vi "Main.vi"() -> ()   [LabVIEW 2013]
doc: "This template is for the Queued Message Handler design pattern.\n\nThe Event Handling Loop generates messages based on user interface actions.\n\nThe Message Handling Loop processes messages generated by the Event Handling Loop, or by other messages. The messages are string values, so new messages can be added easily to the Message Cases case structure in the Message Handling Loop. Each message cluster can also provide an optional value for Message Data, which is a variant that can be converted to whatever message-specific data is required."
uses:
  <vilib>/vision/Image Controls.llb/IMAQ Image.ctl
  Image Processing/Mask ROI FG Enum.ctl
  Message Passing/MsgQ Loops enum.ctl
  System Status/Status FG Enum.ctl
  Globals/Average Sector Data.vi
  controls/UI Data.ctl
  Message Queue/Message Queue.lvlib
  User Event - Stop/User Event - Stop.lvlib
  Image Processing/Image Processing.lvlib
  Common/State Machines/State Machine Lib.lvlib
  Message Passing/Main MsgQ.lvlib
  Common/GUI/GUI.lvlib
  <vilib>/rvi/interface/nirviReadWriteControl/nirviReadWriteControl.xnode
  FGs/FPGA_Reference.ctl
  FPGA Bitfiles/8-Tap8-bitCamera_FPGATarget_8-Tap8-bit_Serial_Server.lvbitx
  <vilib>/rvi/errors/niLvFpgaMergeErrorWithErrorCode.vi
  NiFpgaLv.dll
  <vilib>/rvi/errors/niLvFpgaAdjustHostInterfaceError.vi
panel:
  out "Frames Acquired":u32
  in  "Disable Background Subtraction":bool
  out "Analysis Ticks":u32
  out "Accumulate Ticks":u32
  out "FPGA Display Image":T1(plugin-control)
  out "Right Wingbeat Avg Graph":u8[](graph)
  in  "Start Serial Server":bool=TRUE
  out "Left Wingbeat Avg Graph":u8[](graph)
  in  "Stop Charts":bool
  in  "Wing ROIs":T2
  out "FPGA image info":T5={"Image Type"=0, "Unit"=enum."Undefined", "X Resolution"=2040, "Y Resolution"=1088, "X Step"=1.0, "Y Step"=1.0, "Image Name"="Image"} {"Image Type" items=["Grayscale (U8)", "Grayscale (I16)", "Grayscale (SGL)", "Complex (CSG)", "RGB (U32)", "HSL (U32)", "RGB (U64)", "Grayscale (U16)"]}
  in  "Stream?":bool
  out "FPGA Image":T1
  in  "Test Visual Response":bool
  in  "Test FPGA":bool
  out "Status Update":string="VI Stopped"
  in  "Define Mask":bool
  in  "Acquire Image":bool
  in  "Stop":bool
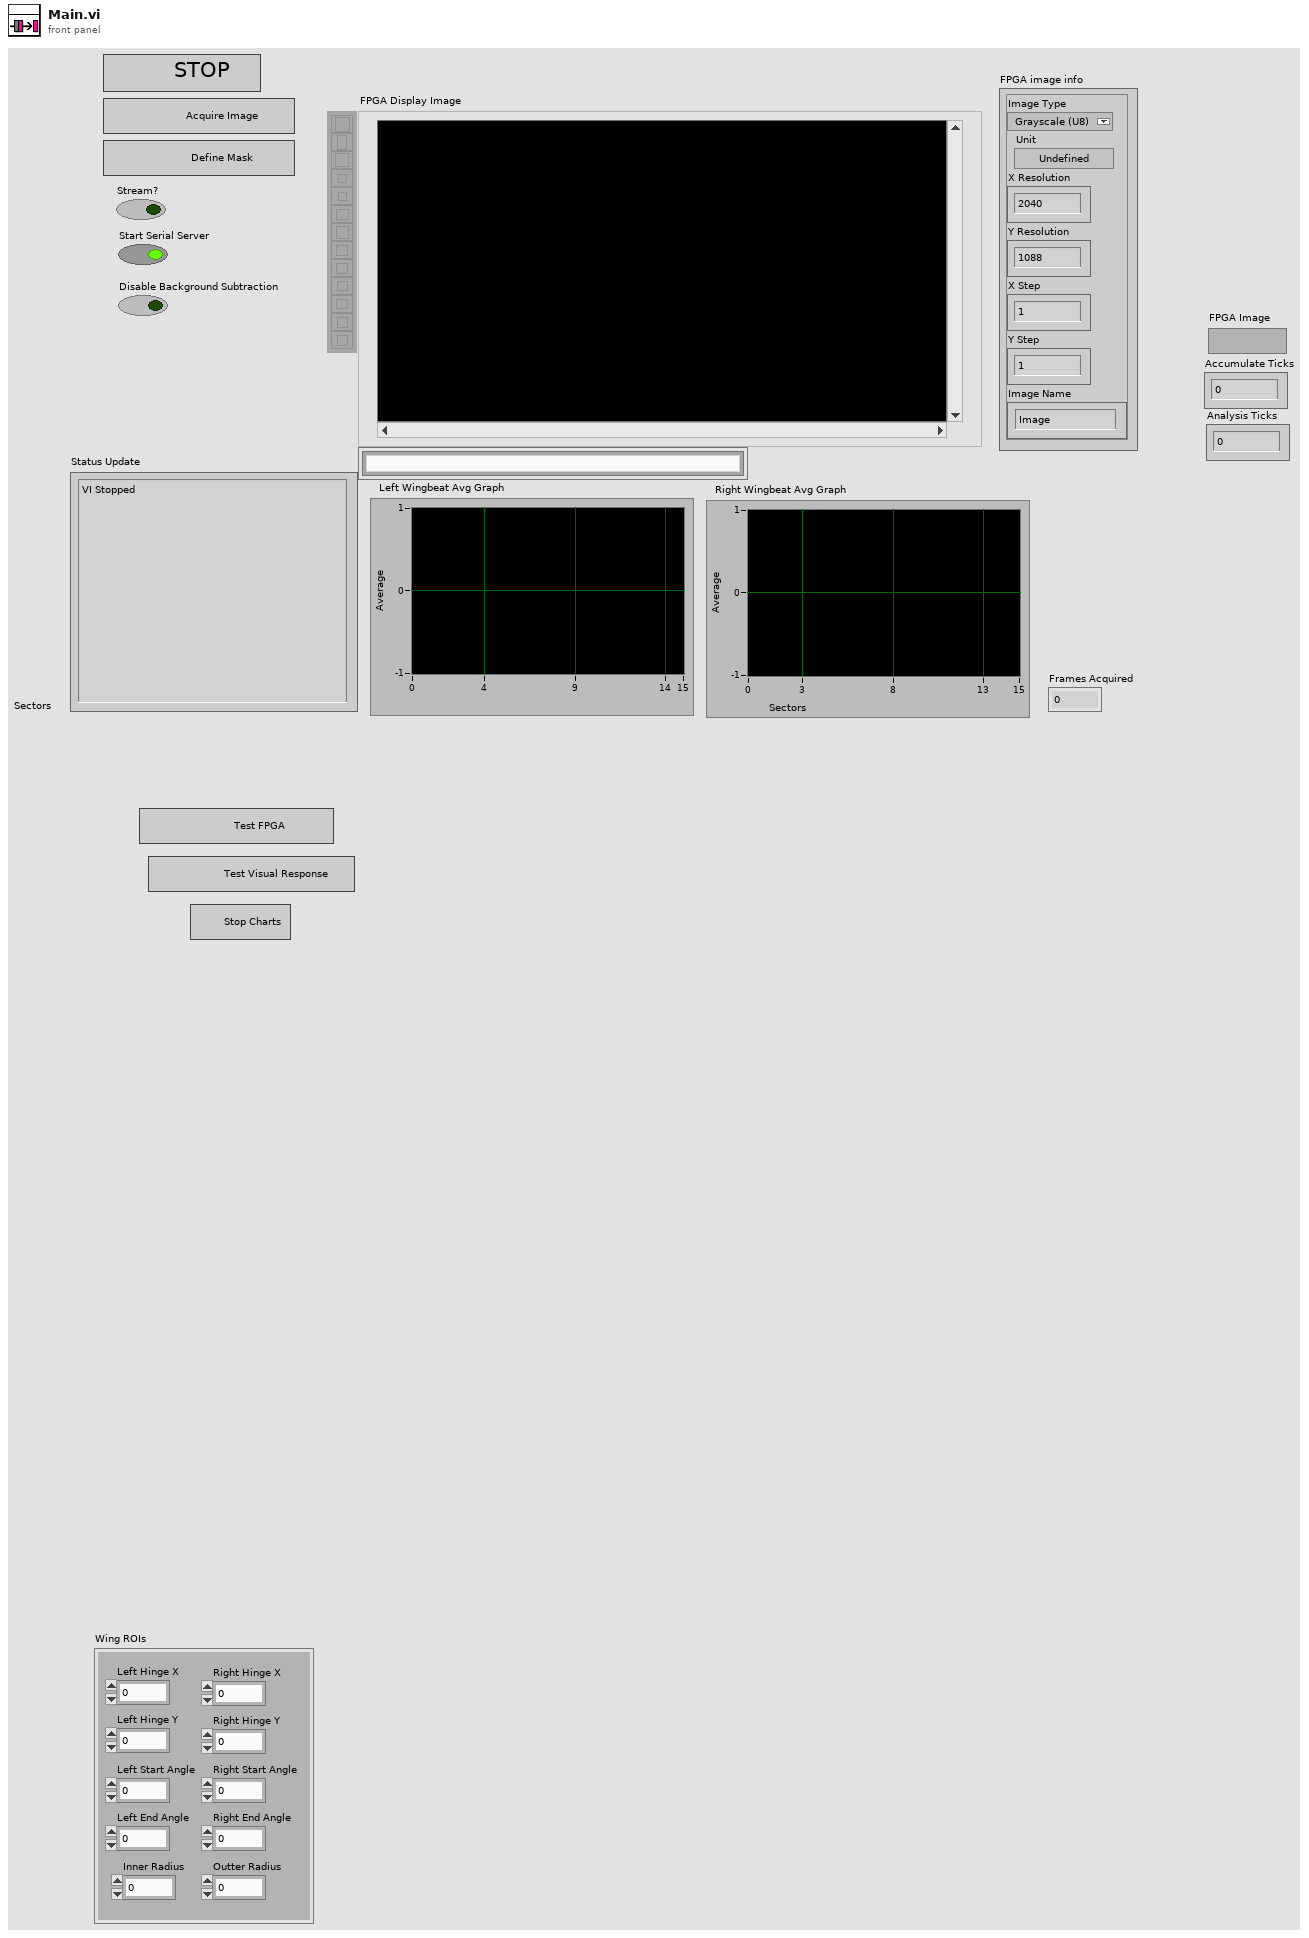
[diagram p1: front panel]
types:
  T1 = typedef "IMAQ Image.ctl" = refnum<image>
  T2 = cluster{"Left Hinge X":u16, "Left Hinge Y":u16, "Inner Radius":u16, "Outter Radius":u16, "Right Hinge X":u16, "Right Hinge Y":u16, "Right Start Angle":i16, "Right End Angle":i16, "Left Start Angle":i16, "Left End Angle":i16}
  T3 = typedef "Image Type" = u32
  T4 = typedef "Image Unit" = enum32{"Undefined", "Angström", "Micrometer", "Millimeter", "Centimeter", "Meter", "Kilometer", "Microinch", "Inch", "Feet", "Nautical miles", "Standard miles", "Steps"}
  T5 = cluster{"Image Type":T3, "Unit":T4, "X Resolution":i32, "Y Resolution":i32, "X Step":sgl, "Y Step":sgl, "Image Name":string}
  T6 = typedef "State Machine Lib.lvlib/STATE cluster.ctl" = cluster{"State":string, "Parameters":variant}
  T7 = typedef "Main MsgQ.lvlib/MsgQ Loops enum.ctl" = enum16{"User Interface", "Image Acq"}
  T8 = typedef "Mask ROI FG Enum.ctl" = enum16{"Read", "Write", "Enable Background", "Disable Background"}
  T9 = typedef "Status FG Enum.ctl" = enum16{"Reset", "Read", "Write"}
  T10 = typedef "FPGA_Reference.ctl" = refnum<k20>
  T11 = typedef "Mask ROI Cluster.ctl" = cluster{"left annulus":T12, "right annulus":T12, "Threshold Range":cluster{"Lower value":dbl, "Upper value":dbl}, "[Avg BG]":u8[], "Number of Sectors":u8, "Left ROI":T13, "Right ROI":T13, "Left Start Angle Duty Cycle":fxp<+,8,0>, "Left End Angle Duty Cycle":fxp<+,8,0>, "Right End Angle Duty Cycle":fxp<+,8,0>, "Right Start Angle Duty Cycle":fxp<+,8,0>, "[Sector ROIs]":T13[]}
  T12 = typedef "IMAQ Circle" = cluster{"Center X":i32, "Center Y":i32, "Inner Radius":i32, "Outer Radius":i32, "Start Angle":dbl, "End Angle":dbl}
  T13 = typedef "ROI Descriptor" = cluster{"Global Rectangle":i32[], "Contours":cluster{"ID":enum32{"External", "Internal"}, "Type":u32, "Coordinates":i32[]}[]}
  T14 = typedef "UI Data.ctl" = cluster{"Boolean <Replace Me>":bool, "Initial Message":string, "Numeric <Replace Me>":dbl, "Acquire Image Ref":refnum<vi>, "Define Mask Ref":refnum<vi>, "Status Update Ref":refnum<vi>, "Stop Button Ref":refnum<vi>, "FPGA Image":T1, "Processed Image":T1, "Left Annulus":cluster{"Center X":i32, "Center Y":i32, "Inner Radius":i32, "Outer Radius":i32, "Start Angle":dbl, "End Angle":dbl}, "Right Annulus":cluster{"Center X":i32, "Center Y":i32, "Inner Radius":i32, "Outer Radius":i32, "Start Angle":dbl, "End Angle":dbl}}
  T15 = typedef "Message Queue.lvlib/All Message Queues.ctl" = cluster{"UI":refnum<queue>}
  T16 = cluster{"Center X":i32, "Center Y":i32, "Inner Radius":i32, "Outer Radius":i32, "Start Angle":dbl, "End Angle":dbl}
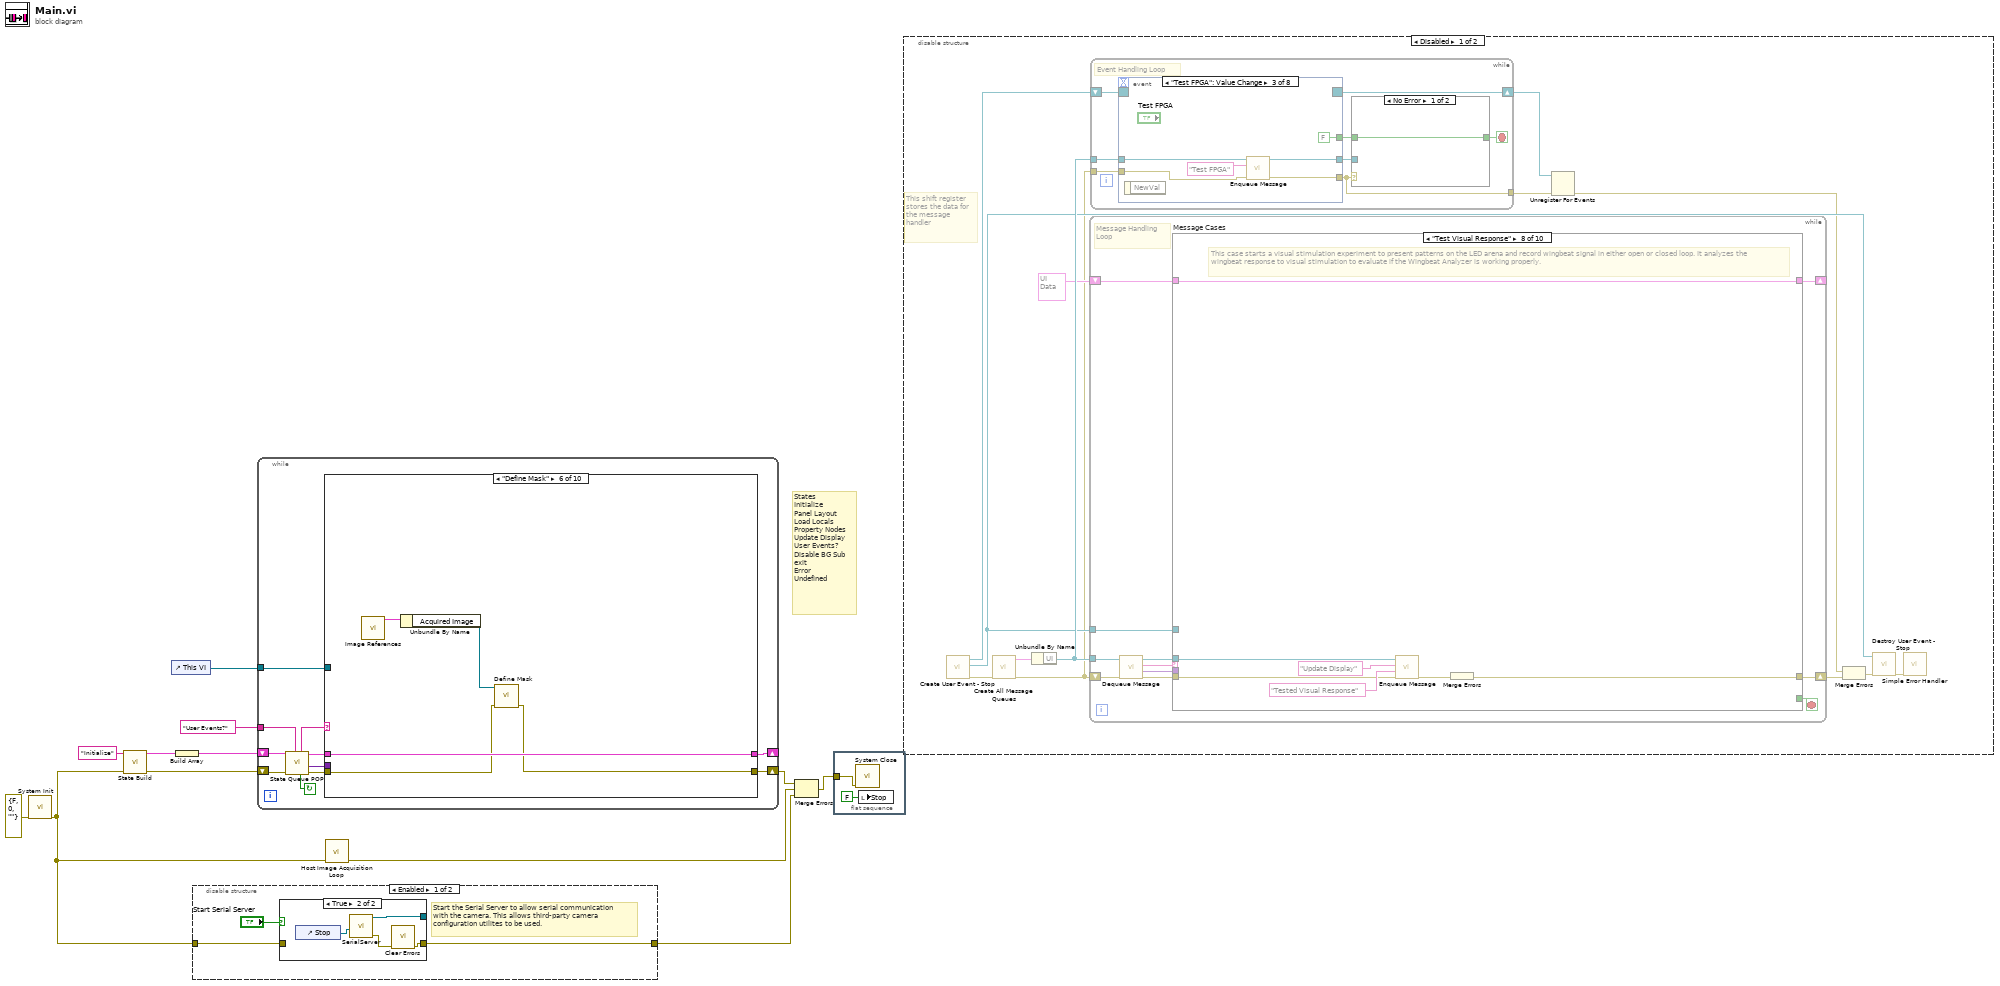
[diagram p0: block diagram]
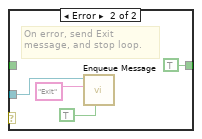
[diagram p4: hidden frame]
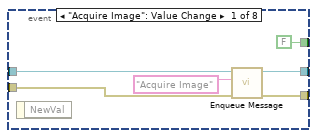
[diagram p5: hidden frame]
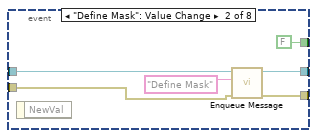
[diagram p6: hidden frame]
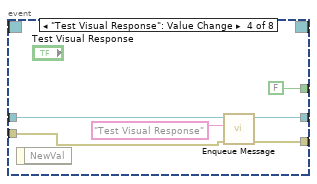
[diagram p7: hidden frame]
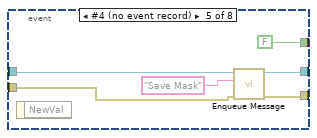
[diagram p8: hidden frame]
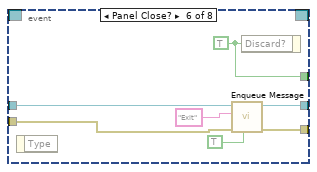
[diagram p9: hidden frame]
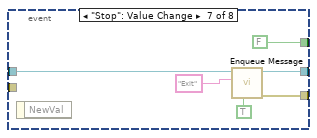
[diagram p10: hidden frame]
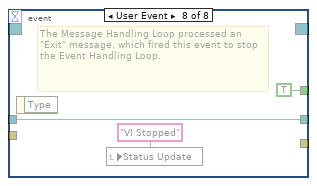
[diagram p11: hidden frame]
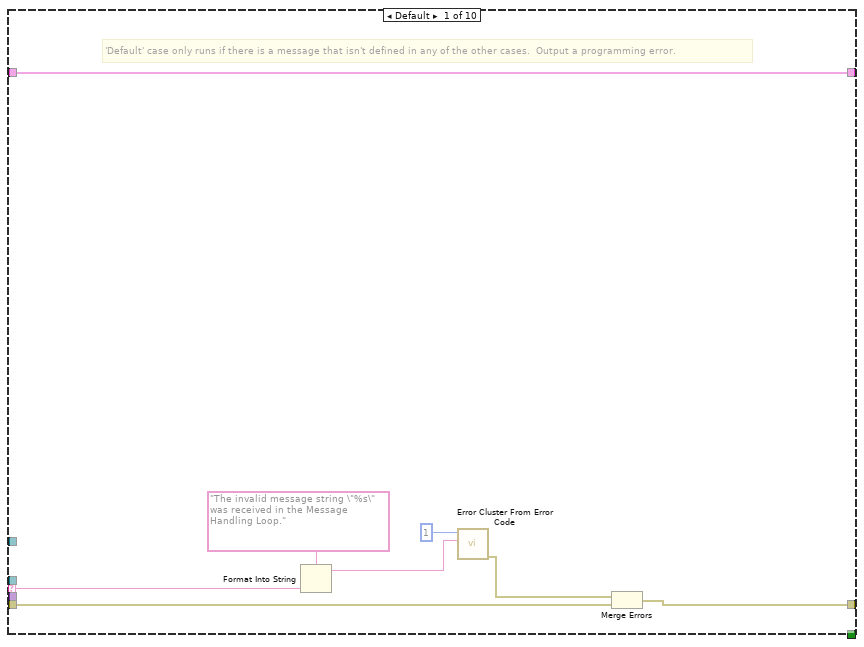
[diagram p12: hidden frame]
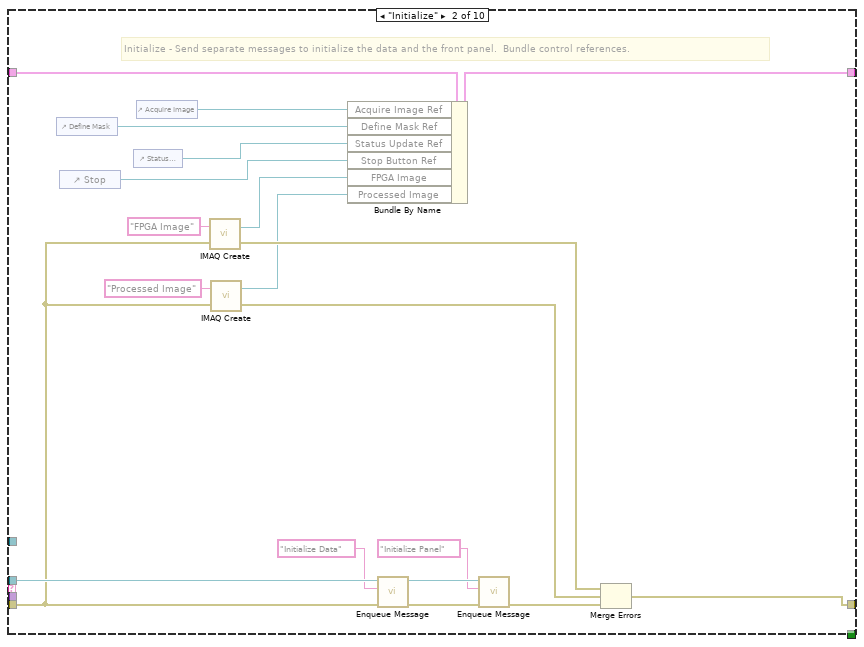
[diagram p13: hidden frame]
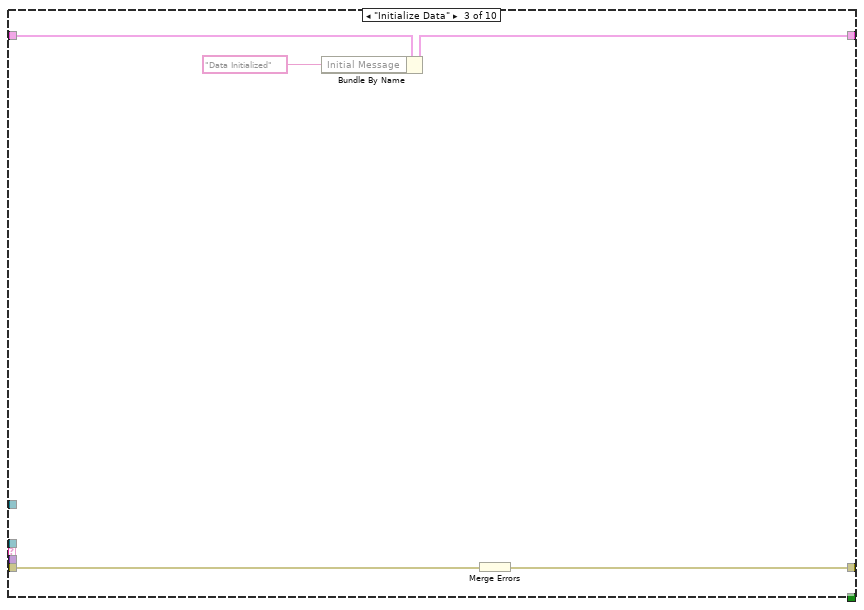
[diagram p14: hidden frame]
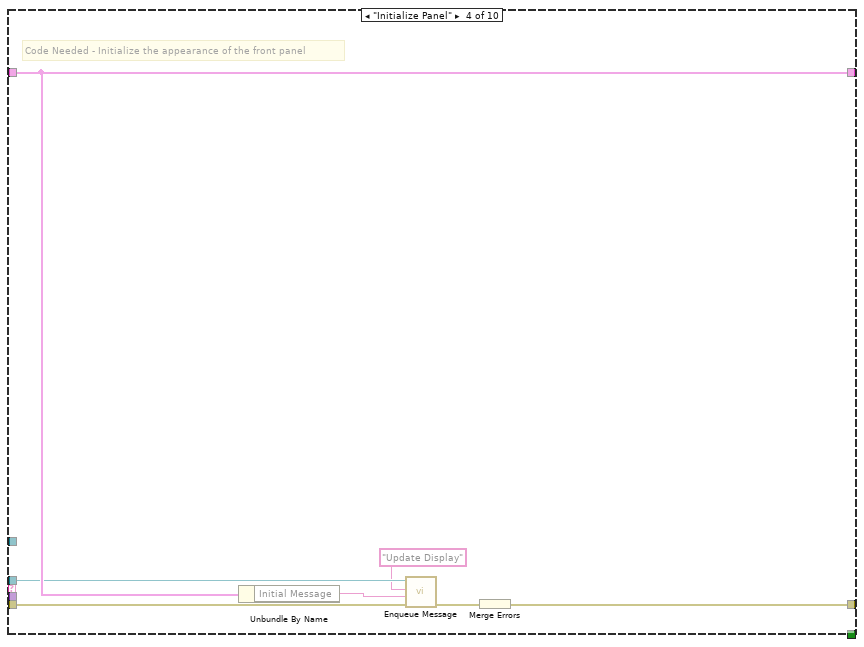
[diagram p15: hidden frame]
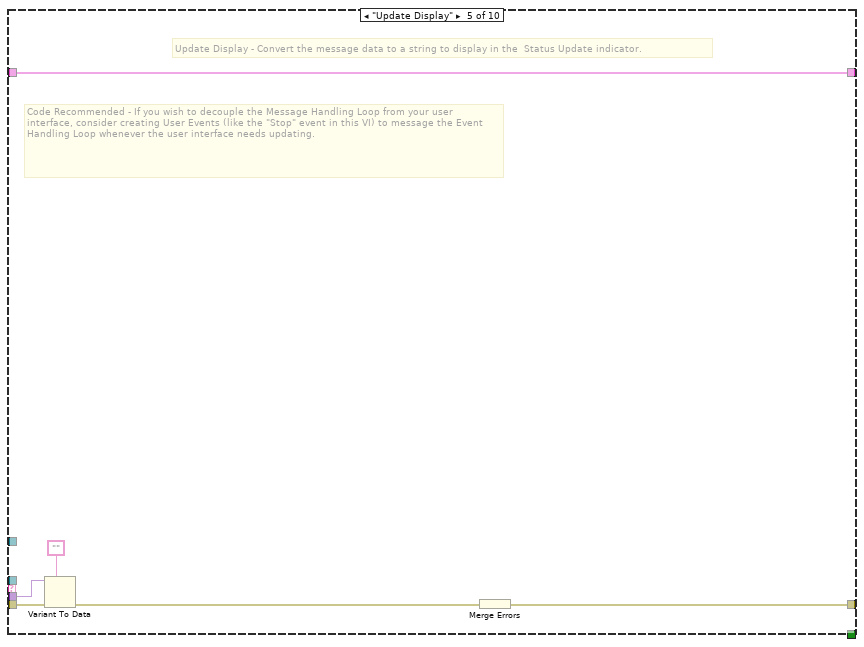
[diagram p16: hidden frame]
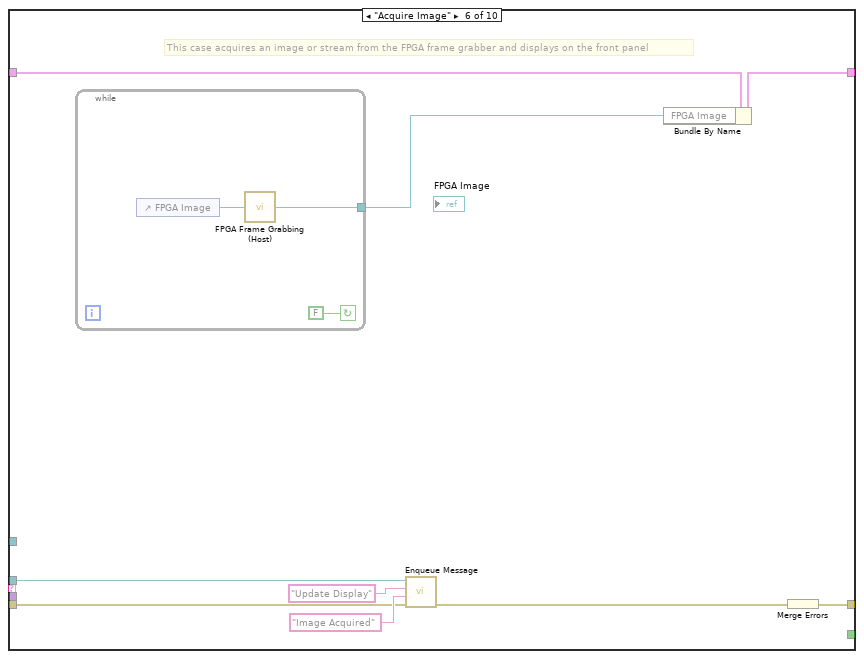
[diagram p17: hidden frame]
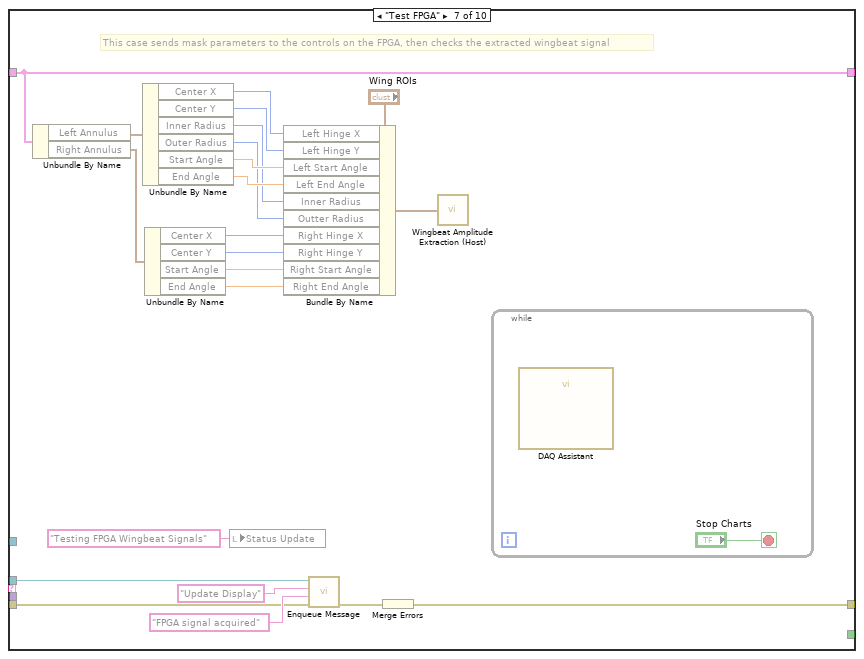
[diagram p18: hidden frame]
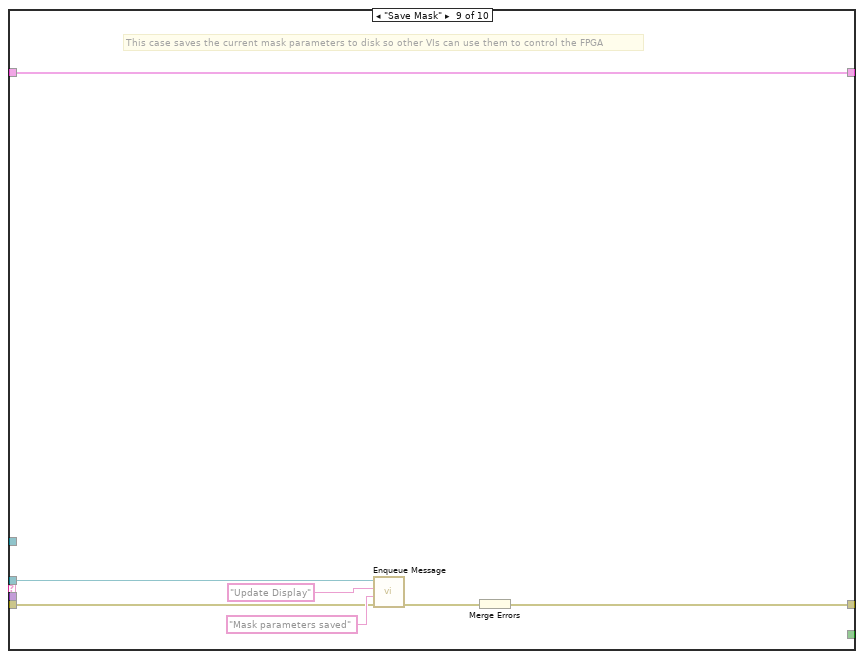
[diagram p19: hidden frame]
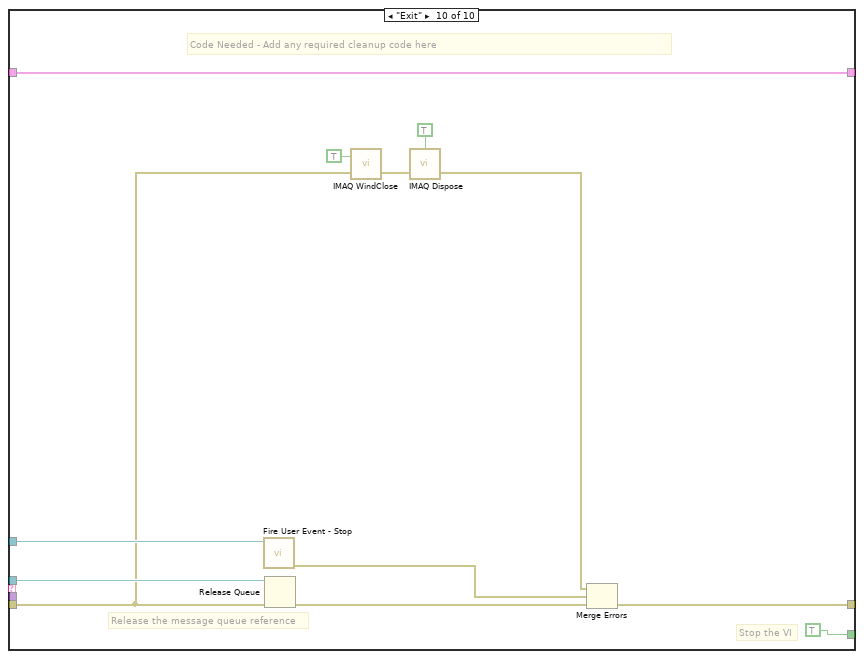
[diagram p20: hidden frame]
diagram:
  # "States\nInitialize\nPanel Layout\nLoad Locals\nProperty Nodes\nUpdate Display\nUser Events?\nDisable BG Sub\nexit\nError\nUndefined"
  n1 = call "System Init.vi"("error in (no error)"=errorcluster {"status"=FALSE, "code"=0, "source"=""}) -> ("error out"=w11:errorcluster)  [unwired: 10 in]
  n2 = call "State Build.vi"("error in (no error)"=w11, "State"="Initialize") -> ("error out"=w7:errorcluster, "State Out"=w9:T6)  [unwired: 8 in]
  n3 = control-ref of="This VI"() -> (w5:refnum<vi>)
  n4 = Build Array(w9) -> (w8:T6[])
  n5 = disable-structure shown="Enabled" {
    disable-tunnel: w11 -> [w14 _]
    disable-tunnel: [w13 _] -> w1
    frame Enabled {
      # "Start the Serial Server to allow serial communication\nwith the camera. This allows third-party camera\nconfiguration utilites to be used."
      n6 = case shown="True" "Start Serial Server" {
        tunnel: [_ w20] -> _
        tunnel: w14 -> [w16 _]
        tunnel: [w16 w18] -> w13
        frame False {
        }
        frame True {
          n7 = control-ref of="Stop"() -> (w19:refnum<vi>)
          n8 = call "SerialServer.vi"("Stop Refnum"=w19) -> ("error out"=w17:errorcluster, "FPGA VI Reference Out"=w20:refnum<k20>)  [unwired: 5 in]
          n9 = call <vilib>:"Clear Errors.vi"("error in (no error)"=w17) -> ("error out"=w18:errorcluster)  [unwired: 6 in]
        }
      }
    }
    frame Disabled {
    }
  }
  n10 = while {
    shift-right: [w25] -> _
    shift-left: w8 -> [w31]
    shift-right: [w23] -> w4
    shift-left: w7 -> [w30]
    tunnel: "User Events?" ("State") -> [w28]
    tunnel: w5 -> [w26]
    stop <- w29 continue-if-true
    n11 = call "State Queue POP.vi"("Default state"=w28, "error in (no error)"=w30, "State que in"=w31) -> ("error out"=w22:errorcluster, "Parameters"=w21:variant, "State que out"=w24:T6[], "Not Exit?"=w29:bool, "State case out"=w27:string)  [unwired: 4 in]
    n12 = case shown="\"Define Mask\"" w27 {
      tunnel: w26 -> [_ _ w42 _ _ _ _ _ _ _]
      tunnel: [w33 w34 w39 w45 w47 w52 w53 w70 w108 w136] -> w25
      tunnel: w24 -> [w33 w37 w39 w45 w47 w52 w53 w69 _ w136]
      tunnel: [w32 w35 w40 w44 w46 w50 w54 w68 w107 w134] -> w23
      tunnel: w22 -> [w32 w36 w41 w44 w46 w51 w65 w67 w109 w118]
      tunnel: w21 -> [_ _ _ _ _ _ w64 w66 _ _]
      frame Default {
      }
      frame "Initialize" {
        n13 = call "State Queue PUSH multiple states no parameters.vi"("States to queue"=string[] ["Panel Layout", "Load Locals", "Property Nodes", "Update Display"], "error in (no error)"=w36, "State que in"=w37) -> ("error out"=w35:errorcluster, "State que out"=w34:T6[])  [unwired: 7 in]
      }
      frame "Panel Layout" {
        # "Reset origin to 0,0"
        n14 = call "Reset all pane origins.vi"("error in (no error"=w41, "Vi Ref In"=w42) -> ("error out"=w40:errorcluster)  [unwired: 8 in, 1 out]
      }
      frame "Load Locals" {
        w43 = FALSE ("Stream?")
        n15 = local write "Stream?"(w43) -> ()
        n16 = local write "Disable Background Subtraction"(w43) -> ()
      }
      frame "Property Nodes" {
      }
      frame "Define Mask" {
        n17 = call "Image References.vi"() -> ("Images"=w49:cluster{"Acquired Image":T1, "Display Image":T1})  [unwired: 10 in, 1 out]
        n18 = Unbundle By Name(w49) -> ("Acquired Image"=w48:T1)
        n19 = call "Define Mask.vi"("error in (no error)"=w51, "FPGA Image"=w48) -> ("error out"=w50:errorcluster)  [unwired: 9 in]
      }
      frame "Disable BG Sub" {
        n20 = Variant To Data(error in=w65, type=FALSE, Variant=w64) -> (data=w62:bool, error out=w59:errorcluster)
        n21 = Select(t=Mask_ROI_FG_Enum."Disable Background" ("Operation"), s=w62, f=Mask_ROI_FG_Enum."Enable Background" ("Operation")) -> (s? t:f=w58:T8)
        n22 = call "Mask ROI FG.vi"("error in (no error)"=w59, "Operation"=w58) -> ("error out"=w55:errorcluster)  [unwired: 8 in, 1 out]
        n23 = call "Send MsgQ.vi"("error in (no error)"=w55, "Message String"="Update Sector Parameters", "Send to MsgQ"=MsgQ_Loops_enum."Image Acq") -> ("error out"=w54:errorcluster)  [unwired: 8 in]
      }
      frame "User Events?" {
        n24 = event shown="[0] Timeout" {
          selector: _ -> [_ _ _ _ _ _]
          dyn-events: _ -> [_ _ _ _ _ _]
          timeout: 200 -> [_ _ _ _ _ _]
          tunnel: [w73 w83 w86 w93 w99 w102] -> w70
          tunnel: w69 -> [w74 w83 w86 w95 w101 w105]
          tunnel: [w75 w80 w87 w92 w98 w103] -> w68
          tunnel: w67 -> [w76 w81 w88 w94 w100 w104]
          tunnel: w66 -> [_ _ _ _ _ _]
          event Timeout {
            n25 = event-data() -> ()  [unwired: 1 in, 3 out]
            n26 = disable-structure shown="Disabled" {
              frame Disabled {
                n27 = call "FPGA Reference FG.vi"() -> ("FPGA VI Reference Out"=w79:T10)  [unwired: 11 in]
                n28 = xnode "Read/Write Control"("FPGA VI Reference In"=w79) -> ("Accumulate Ticks"=→"Accumulate Ticks", "Analysis Ticks"=→"Analysis Ticks":u32)  [unwired: 1 in, 2 out]
              }
              frame Enabled {
              }
            }
            n29 = call "State Queue PUSH.vi"("State case"="Update Display", "error in (no error)"=w76, "State que in"=w74) -> ("error out"=w75:errorcluster, "State que out"=w73:T6[])  [unwired: 7 in]
          }
          event "Acquire Image": Value Change {
            n30 = event-data() -> ()  [unwired: 1 in, 6 out]
            n31 = call "Send MsgQ.vi"("error in (no error)"=w81, "Message String"="Acquire Single Image", "Send to MsgQ"=MsgQ_Loops_enum."Image Acq") -> ("error out"=w80:errorcluster)  [unwired: 8 in]
          }
          event "Stream?": Value Change {
            n32 = event-data() -> ("NewVal"=w85:bool)  [unwired: 1 in, 5 out]
            n33 = call "Send MsgQ.vi"("error in (no error)"=w88, "Data In"=w85, "Message String"="Stream Image", "Send to MsgQ"=MsgQ_Loops_enum."Image Acq") -> ("error out"=w87:errorcluster)  [unwired: 7 in]
          }
          event "Define Mask": Value Change {
            n34 = event-data() -> ()  [unwired: 1 in, 6 out]
            n35 = call "State Queue PUSH.vi"("State case"="Define Mask", "error in (no error)"=w94, "State que in"=w95) -> ("error out"=w92:errorcluster, "State que out"=w93:T6[])  [unwired: 7 in]
          }
          event "Disable Background Subtraction": Value Change {
            n36 = event-data() -> ("NewVal"=w96:bool)  [unwired: 1 in, 5 out]
            n37 = call "State Queue PUSH.vi"("State case"="Disable BG Sub", "error in (no error)"=w100, "Parameters"=w96, "State que in"=w101) -> ("error out"=w98:errorcluster, "State que out"=w99:T6[])  [unwired: 6 in]
          }
          event "Stop": Value Change {
            n38 = event-data() -> ()  [unwired: 1 in, 6 out]
            n39 = call "State Queue PUSH.vi"("State case"="exit", "error in (no error)"=w104, "State que in"=w105) -> ("error out"=w103:errorcluster, "State que out"=w102:T6[])  [unwired: 7 in]
          }
        }
      }
      frame "exit" {
        n40 = call "Broadcast Exit.vi"("error in"=w109) -> ("error out"=w107:errorcluster)  [unwired: 10 in]
        n41 = call "Queue EXIT state.vi"() -> ("Exit State Q"=w108:T6[])  [unwired: 1 in]
      }
      frame "Update Display" {
        n42 = call "Image References.vi"() -> ("Images"=w114:cluster{"Acquired Image":T1, "Display Image":T1})  [unwired: 10 in, 1 out]
        n43 = call "Status FG.vi"("Operation"=Status_FG_Enum."Read") -> ("Status Out"=→"Status Update":string)  [unwired: 9 in, 1 out]
        n44 = call "Mask ROI FG.vi"("Operation"=Mask_ROI_FG_Enum."Read") -> ("Mask ROI Out"=w131:T11)  [unwired: 9 in, 1 out]
        n45 = Unbundle By Name(w114) -> ("Acquired Image"=w113:T1, "Display Image"=w112:T1)
        n46 = Unbundle By Name(w131) -> ("Number of Sectors"=w128:u8)
        n47 = global read "Average Sector Data.vi" "# of Frames Acquired"() -> (→"Frames Acquired":u32)
        n48 = global read "Average Sector Data.vi" "[Average Sector Data]"() -> (w133:u8[])
        n49 = call "Overlay Image with Sector ROI.vi"("FPGA Display Image In"=w112, "error in"=w118, "FPGA Image"=w113) -> ("error out"=w117:errorcluster, "FPGA Display Image Out"=→"FPGA Display Image":T1)  [unwired: 7 in]
        n50 = call "IMAQ GetImageInfo"("error in (no error)"=w117, "Image"=w113) -> ("error out"=w135:errorcluster, "X Step"=w123:sgl, "Y Resolution"=w122:i32, "X Resolution"=w121:i32, "Y Step"=w124:sgl, "Unit"=w120:T4, "Image Name"=w125:string, "Image Type"=w119:T3)  [unwired: 2 in]
        n51 = Split 1D Array(array=w133, index=w128) -> (first subarray=→"Left Wingbeat Avg Graph":u8[], second subarray=→"Right Wingbeat Avg Graph":u8[])
        n52 = local read "FPGA image info"() -> (w127:T5)
        n53 = Bundle By Name(cluster=w127, "Image Type"=w119, "Unit"=w120, "X Resolution"=w121, "Y Resolution"=w122, "X Step"=w123, "Y Step"=w124, "Image Name"=w125) -> (→"FPGA image info":T5)
        n54 = call <vilib>:"Clear Errors.vi"("error in (no error)"=w135) -> ("error out"=w134:errorcluster)  [unwired: 6 in]
      }
    }
  }
  n55 = call "Host Image Acquisition Loop.vi"("error in"=w11) -> ("error out"=w3:errorcluster)  [unwired: 10 in]
  n56 = Merge Errors(w4, w3, w1) -> (w2:errorcluster)
  n57 = flat-sequence {
    tunnel: w2 -> [w138]
    frame #0 {
      n58 = call "System Close.vi"("error in (no error)"=w138) -> ()  [unwired: 10 in, 1 out]
      n59 = local write "Stop"(FALSE ("Stop")) -> ()
    }
  }
  n60 = disable-structure shown="Disabled" {
    frame Disabled {
      # "This shift register\nstores the data for the message handler"
      n61 = call "Create User Event - Stop.vi"() -> ("error out"=w147:errorcluster, "User Event - Stop"=w144:refnum<user-event>, "Stop Event Registration Refnum"=w148:refnum<event-registration>)  [unwired: 9 in]
      n62 = call "Create All Message Queues.vi"("error in (no error)"=w147) -> ("error out"=w139:errorcluster, "Message Queues out"=w151:T15)  [unwired: 9 in]
      n63 = Unbundle By Name(w151) -> ("UI"=w149:refnum<queue>)
      n64 = while {
        tunnel: w149 -> [w211]
        shift-right: [w220] -> _
        shift-left: T14 {"Boolean <Replace Me>"=TRUE, "Initial Message"="", "Numeric <Replace Me>"=0.0, "Acquire Image Ref"=refnum, "Define Mask Ref"=refnum, "Status Update Ref"=refnum, "Stop Button Ref"=refnum, "FPGA Image"=refnum, "Processed Image"=refnum, "Left Annulus"={"Center X"=0, "Center Y"=0, "Inner Radius"=0, "Outer Radius"=0, "Start Angle"=0.0, "End Angle"=0.0}, "Right Annulus"={"Center X"=0, "Center Y"=0, "Inner Radius"=0, "Outer Radius"=0, "Start Angle"=0.0, "End Angle"=0.0}} ("Data Cluster") -> [w221]
        tunnel: w144 -> [w217]
        shift-right: [w218] -> w150
        shift-left: w139 -> [w216]
        stop <- w219 stop-if-true
        # "Message Handling Loop"
        n65 = call "Dequeue Message.vi"("error in (no error)"=w216, "Message Queue"=w211) -> ("error out"=w215:errorcluster, "Message Data"=w213:variant, "Message"=w214:string, "dup Message Queue"=w212:refnum<queue>)  [unwired: 6 in]
        n66 = case "Message Cases" shown="\"Test Visual Response\"" w214 {
          selector: w214 -> [w227 _ _ _ _ _ _ _ _ _]
          tunnel: w212 -> [_ w247 _ w258 _ w275 w298 w306 w314 w330]
          tunnel: w215 -> [w224 w232 w254 w259 w266 w270 w299 w307 w312 w319]
          tunnel: [w222 w234 w250 w260 w267 w277 w297 w305 w317 w326] -> w218
          tunnel: w221 -> [w229 w244 w253 w261 w268 w272 w296 w311 w318 w329]
          tunnel: [w229 w243 w252 w261 w268 w271 w296 w311 w318 w329] -> w220
          tunnel: [_ _ _ _ _ _ _ _ _ TRUE] -> w219
          tunnel: w213 -> [_ _ _ _ w265 _ _ _ _ _]
          tunnel: w217 -> [_ _ _ _ _ _ _ _ _ w325]
          frame Default {
            # "'Default' case only runs if there is a message that isn't defined in any of the other cases.  Output a programming error."
            n67 = Format Into String(format string="The invalid message string \"%s\" was received in the Message Handling Loop." ("Unknown Message Error Text"), w227) -> (resulting string=w225:string)  [unwired: 2 in, 1 out]
            n68 = call <vilib>:"Error Cluster From Error Code.vi"("error message (\"\")"=w225, "error code (0)"=1) -> ("error out"=w223:errorcluster)  [unwired: 7 in]
            n69 = Merge Errors(w223, w224) -> (w222:errorcluster)
          }
          frame "Initialize" {
            # "Initialize - Send separate messages to initialize the data and the front panel.  Bundle control references."
            n70 = control-ref of="Define Mask"() -> (w241:refnum<vi>)
            n71 = control-ref of="Stop"() -> (w239:refnum<vi>)
            n72 = control-ref of="Status Update"() -> (w240:refnum<vi>)
            n73 = control-ref of="Acquire Image"() -> (w242:refnum<vi>)
            n74 = call "IMAQ Create"("Image Name"="FPGA Image", "error in (no error)"=w232) -> ("New Image"=w237:T1, "error out"=w233:errorcluster)  [unwired: 3 in]
            n75 = call "IMAQ Create"("Image Name"="Processed Image", "error in (no error)"=w232) -> ("New Image"=w230:T1, "error out"=w231:errorcluster)  [unwired: 3 in]
            n76 = Bundle By Name(cluster=w244, "Acquire Image Ref"=w242, "Define Mask Ref"=w241, "Status Update Ref"=w240, "Stop Button Ref"=w239, "FPGA Image"=w237, "Processed Image"=w230) -> (w243:T14)
            n77 = call "Enqueue Message.vi"("error in (no error)"=w232, "Message"="Initialize Data", "Message Queue"=w247) -> ("error out"=w249:errorcluster, "dup Message Queue"=w248:refnum<queue>)  [unwired: 7 in]
            n78 = call "Enqueue Message.vi"("error in (no error)"=w249, "Message"="Initialize Panel", "Message Queue"=w248) -> ("error out"=w235:errorcluster)  [unwired: 7 in, 1 out]
            n79 = Merge Errors(w233, w231, w235) -> (w234:errorcluster)
          }
          frame "Initialize Data" {
            n80 = Bundle By Name(cluster=w253, "Initial Message"="Data Initialized") -> (w252:T14)
            n81 = Merge Errors(w254) -> (w250:errorcluster)
          }
          frame "Initialize Panel" {
            # "Code Needed - Initialize the appearance of the front panel"
            n82 = Unbundle By Name(w261) -> ("Initial Message"=w255:string)
            n83 = call "Enqueue Message.vi"("error in (no error)"=w259, "Message Data"=w255, "Message"="Update Display", "Message Queue"=w258) -> ("error out"=w257:errorcluster)  [unwired: 6 in, 1 out]
            n84 = Merge Errors(w257) -> (w260:errorcluster)
          }
          frame "Update Display" {
            # "Code Recommended - If you wish to decouple the Message Handling Loop from your user interface, consider creating User Events (like the \"Stop\" event in this VI) to message the Event Handling Loop whenever the user interface needs updating."
            # "Update Display - Convert the message data to a string to display in the  Status Update indicator."
            n85 = Variant To Data(error in=w266, type="", Variant=w265) -> (data=w262:string, error out=w263:errorcluster)
            n86 = Merge Errors(w263) -> (w267:errorcluster)
          }
          frame "Acquire Image" {
            # "This case acquires an image or stream from the FPGA frame grabber and displays on the front panel"
            n87 = while {
              tunnel: [w280] -> w269
              stop <- FALSE continue-if-true
              n88 = control-ref of="FPGA Image"() -> (w279:refnum<vi>)
              n89 = call "FPGA Frame Grabbing (Host).vi"("Ctl Refnum"=w279) -> ("Image"=w280:T1)
            }
            n90 = call "Enqueue Message.vi"("error in (no error)"=w270, "Message Data"="Image Acquired" ("\"Do Something\" button pressed"), "Message"="Update Display", "Message Queue"=w275) -> ("error out"=w276:errorcluster)  [unwired: 6 in, 1 out]
            n91 = Bundle By Name(cluster=w272, "FPGA Image"=w269) -> (w271:T14)
            n92 = Merge Errors(w276) -> (w277:errorcluster)
          }
          frame "Test FPGA" {
            # "This case sends mask parameters to the controls on the FPGA, then checks the extracted wingbeat signal"
            n93 = Unbundle By Name(w296) -> ("Left Annulus"=w295:T16, "Right Annulus"=w294:T16)
            n94 = Unbundle By Name(w295) -> ("Center X"=w292:i32, "Center Y"=w291:i32, "Inner Radius"=w288:i32, "Outer Radius"=w287:i32, "Start Angle"=w290:dbl, "End Angle"=w289:dbl)
            n95 = Unbundle By Name(w294) -> ("Center X"=w286:i32, "Center Y"=w285:i32, "Start Angle"=w284:dbl, "End Angle"=w283:dbl)
            n96 = local write "Status Update"("Testing FPGA Wingbeat Signals" ("Status Update")) -> ()
            n97 = Bundle By Name(cluster="Wing ROIs", "Left Hinge X"=w292, "Left Hinge Y"=w291, "Left Start Angle"=w290, "Left End Angle"=w289, "Inner Radius"=w288, "Outter Radius"=w287, "Right Hinge X"=w286, "Right Hinge Y"=w285, "Right Start Angle"=w284, "Right End Angle"=w283) -> (w282:T2)
            n98 = call "Enqueue Message.vi"("error in (no error)"=w299, "Message Data"="FPGA signal acquired" ("\"Do Something\" button pressed"), "Message"="Update Display", "Message Queue"=w298) -> ("error out"=w302:errorcluster)  [unwired: 6 in, 1 out]
            n99 = Merge Errors(w302) -> (w297:errorcluster)
            n100 = call "Wingbeat Amplitude Extraction (Host).vi"("Wing ROIs"=w282) -> ()  [unwired: 1 in]
            n101 = while {
              stop <- "Stop Charts" stop-if-true
              n102 = call "DAQ Assistant"() -> ("data"=w303:dynamicdata)  [unwired: 17 in, 2 out]
            }
          }
          frame "Test Visual Response" {
            # "This case starts a visual stimulation experiment to present patterns on the LED arena and record wingbeat signal in either open or closed loop. It analyzes the wingbeat response to visual stimulation to evaluate if the Wingbeat Analyzer is working properly."
            n103 = call "Enqueue Message.vi"("error in (no error)"=w307, "Message Data"="Tested Visual Response" ("\"Do Something\" button pressed"), "Message"="Update Display", "Message Queue"=w306) -> ("error out"=w310:errorcluster)  [unwired: 6 in, 1 out]
            n104 = Merge Errors(w310) -> (w305:errorcluster)
          }
          frame "Save Mask" {
            # "This case saves the current mask parameters to disk so other VIs can use them to control the FPGA"
            n105 = call "Enqueue Message.vi"("error in (no error)"=w312, "Message Data"="Mask parameters saved" ("\"Do Something Else\" button pressed"), "Message"="Update Display", "Message Queue"=w314) -> ("error out"=w313:errorcluster)  [unwired: 6 in, 1 out]
            n106 = Merge Errors(w313) -> (w317:errorcluster)
          }
          frame "Exit" {
            # "Stop the VI"
            # "Release the message queue reference"
            # "Code Needed - Add any required cleanup code here"
            n107 = call "Fire User Event - Stop.vi"("User Event - Stop"=w325) -> ("error out"=w324:errorcluster)  [unwired: 10 in]
            n108 = Release Queue(queue=w330, error in (no error)=w319) -> (error out=w327:errorcluster)  [unwired: 1 in, 2 out]
            n109 = call "IMAQ WindClose"("Close All Windows (False)"=TRUE, "error in (no error)"=w319) -> ("error out"=w321:errorcluster)  [unwired: 4 in]
            n110 = call "IMAQ Dispose"("All Images? (No)"=TRUE, "error in (no error)"=w321) -> ("error out"=w320:errorcluster)  [unwired: 4 in]
            n111 = Merge Errors(w320, w324, w327) -> (w326:errorcluster)
          }
        }
      }
      n112 = while {
        tunnel: w149 -> [w159]
        tunnel: [w155] -> w142
        shift-right: [w153] -> w141
        shift-left: w148 -> [w154]
        tunnel: w139 -> [w152]
        stop <- w157 stop-if-true
        # "Event Handling Loop"
        n113 = event shown="[2] \"Test FPGA\": Value Change" {
          selector: w154 -> [_ _ _ _ _ _ _ _]
          dyn-events: [_ _ _ _ _ _ _ _] -> w153
          timeout: _ -> [_ _ _ _ _ _ _ _]
          tunnel: [FALSE ("Discard?") FALSE ("Discard?") FALSE ("Discard?") FALSE ("Discard?") FALSE ("Discard?") w201 FALSE ("Discard?") TRUE ("Discard?")] -> w158
          tunnel: w159 -> [w170 w176 w182 w187 w192 w200 w207 w210]
          tunnel: [w169 w174 w179 w184 w189 w199 w206 _] -> w155
          tunnel: [w168 w175 w178 w186 w191 w198 w204 w210] -> w156
          tunnel: w152 -> [w166 w172 w180 w183 w190 w195 _ _]
          event "Acquire Image": Value Change {
            n114 = event-data() -> ()  [unwired: 1 in, 1 out]
            n115 = call "Enqueue Message.vi"("error in (no error)"=w166, "Message"="Acquire Image", "Message Queue"=w170) -> ("error out"=w169:errorcluster, "dup Message Queue"=w168:refnum<queue>)  [unwired: 7 in]
          }
          event "Define Mask": Value Change {
            n116 = event-data() -> ()  [unwired: 1 in, 1 out]
            n117 = call "Enqueue Message.vi"("error in (no error)"=w172, "Message"="Define Mask", "Message Queue"=w176) -> ("error out"=w174:errorcluster, "dup Message Queue"=w175:refnum<queue>)  [unwired: 7 in]
          }
          event "Test FPGA": Value Change {
            n118 = event-data() -> ()  [unwired: 1 in, 1 out]
            n119 = call "Enqueue Message.vi"("error in (no error)"=w180, "Message"="Test FPGA", "Message Queue"=w182) -> ("error out"=w179:errorcluster, "dup Message Queue"=w178:refnum<queue>)  [unwired: 7 in]
          }
          event "Test Visual Response": Value Change {
            n120 = event-data() -> ()  [unwired: 1 in, 1 out]
            n121 = call "Enqueue Message.vi"("error in (no error)"=w183, "Message"="Test Visual Response", "Message Queue"=w187) -> ("error out"=w184:errorcluster, "dup Message Queue"=w186:refnum<queue>)  [unwired: 7 in]
          }
          event #4 (no event record) {
            n122 = event-data() -> ()  [unwired: 1 in, 1 out]
            n123 = call "Enqueue Message.vi"("error in (no error)"=w190, "Message"="Save Mask", "Message Queue"=w192) -> ("error out"=w189:errorcluster, "dup Message Queue"=w191:refnum<queue>)  [unwired: 7 in]
          }
          event Panel Close? {
            w201 = TRUE ("Discard?")
            n124 = event-data() -> ()  [unwired: 1 in, 1 out]
            n125 = call "Enqueue Message.vi"("Priority Message? (F)"=TRUE, "error in (no error)"=w195, "Message"="Exit", "Message Queue"=w200) -> ("error out"=w199:errorcluster, "dup Message Queue"=w198:refnum<queue>)  [unwired: 6 in]
            n126 = event-data("Discard?"=w201) -> ()  [unwired: 1 in, 1 out]
          }
          event "Stop": Value Change {
            n127 = event-data() -> ()  [unwired: 1 in, 1 out]
            n128 = call "Enqueue Message.vi"("Priority Message? (F)"=TRUE, "Message"="Exit", "Message Queue"=w207) -> ("error out"=w206:errorcluster, "dup Message Queue"=w204:refnum<queue>)  [unwired: 7 in]
          }
          event User Event {
            # "The Message Handling Loop processed an \"Exit\" message, which fired this event to stop the Event Handling Loop."
            n129 = event-data() -> ()  [unwired: 1 in, 1 out]
            n130 = local write "Status Update"("VI Stopped" ("VI Stopped")) -> ()
          }
        }
        n131 = case shown="No Error" w155 {
          tunnel: [w160 TRUE ("Discard?")] -> w157
          tunnel: w158 -> [w160 _]
          tunnel: w156 -> [_ w163]
          frame No Error {
          }
          frame Error {
            # "On error, send Exit message, and stop loop."
            n132 = call "Enqueue Message.vi"("Priority Message? (F)"=TRUE, "Message"="Exit", "Message Queue"=w163) -> ()  [unwired: 7 in, 2 out]
          }
        }
      }
      n133 = Unregister For Events(event registration refnum=w141, error in=w142) -> (error out=w143:errorcluster)
      n134 = Merge Errors(w143, w150) -> (w145:errorcluster)
      n135 = call "Destroy User Event - Stop.vi"("error in (no error)"=w145, "User Event - Stop"=w144) -> ("error out"=w146:errorcluster)  [unwired: 9 in]
      n136 = call <vilib>:"Simple Error Handler.vi"("error in (no error)"=w146) -> ()  [unwired: 4 in, 5 out]
    }
    frame Enabled {
    }
  }
